vi "Log.vi"(8 "error in (no error)":errorcluster, 9 "Filename":string, 10 "New Log":string, 11 "Log In":string) -> (3 "Log out":string)   [LabVIEW 2021]
doc: "<b>_______________________________________________________________</b>\n** Author: Juan José Villacorta\n** LabVIEW wrapper for C library <b> wiringPi </b>,\n** https://github.com/WiringPi/WiringPi\n<b>_______________________________________________________________</b>"
uses:
  <vilib>/Utility/error.llb/DialogType.ctl
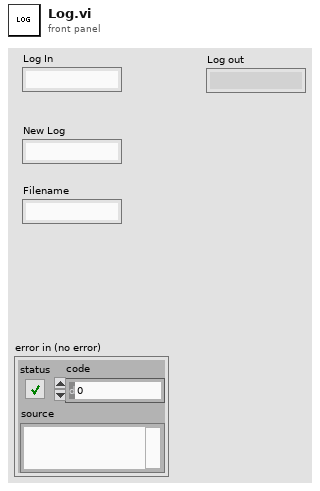
[diagram p1: front panel]
types:
  T1 = typedef "DialogType.ctl" = u16
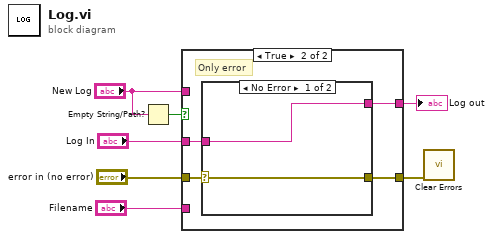
[diagram p0: block diagram]
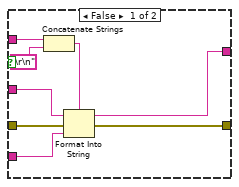
[diagram p2: hidden frame]
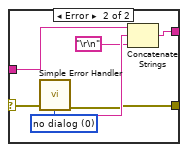
[diagram p3: hidden frame]
diagram:
  n1 = Empty String/Path?(string/path="New Log") -> (empty?=w3:bool)
  n2 = case shown="True" w3 {
    tunnel: [w15 w18] -> w7
    tunnel: [w14 w16] -> w1
    tunnel: "error in (no error)" -> [w13 w19]
    tunnel: "Filename" -> [w12 _]
    tunnel: "New Log" -> [w11 _]
    tunnel: "Log In" -> [w10 w17]
    frame False {
      n3 = Concatenate Strings(w11, "\r\n") -> (w9:string)
      n4 = Format Into String(format string=w9, initial string=w10, error in=w13, w12) -> (resulting string=w15:string, error out=w14:errorcluster)
    }
    frame True {
      # "Only error"
      n5 = case shown="No Error" w19 {
        selector: w19 -> [w20 w27]
        tunnel: [w21 w25] -> w18
        tunnel: w17 -> [w21 w28]
        tunnel: [w20 w22] -> w16
        frame No Error {
        }
        frame Error {
          w26 = T1 0 items=["no dialog", "OK message", "continue or stop message", "OK message + warnings", "continue/stop + warnings"] ("type of dialog (OK msg:1)")
          n6 = call <vilib>:"Simple Error Handler.vi"("type of dialog (OK msg:1)"=w26, "error in (no error)"=w27) -> ("error out"=w22:errorcluster, "message"=w24:string)  [unwired: 3 in, 3 out]
          n7 = Concatenate Strings(w28, w24, "\r\n") -> (w25:string)
        }
      }
    }
  }
  "Log out" <- w7
  n8 = call <vilib>:"Clear Errors.vi"("error in (no error)"=w1) -> ()  [unwired: 5 in, 2 out]
